vi "Migrate v1 Data.vi"(8 "error in (no error)":errorcluster, 11 "Data Folder":path) -> (0 "error out":errorcluster, 3 "migrated?":bool)   [LabVIEW 2024]
doc: "Converts a version-1 data folder to the schema-version-2 layout (see Documentation/Sample Data/README.md). Does nothing and returns migrated? = FALSE when Projects.ini is missing or already carries [_Meta] Schema Version = 2. Otherwise: (1) every *.ini file is copied into a new subfolder Backup v1 YYYY-MM-DD HHMMSS - if that fails the VI stops with the error and changes nothing; (2) Projects.ini is read: each section except [Default] becomes a project with a new GUID (Active TRUE, Sort Order in file order) and its Task_n keys become tasks with new GUIDs (Active from the ::Active / ::Inactive suffix); [Default] becomes Settings.ini [Default Tasks] Task_0..n; (3) every YYYY-MM.ini month file is read - entries keep their GUID, project and task names are resolved to IDs and missing ones are created with Active FALSE; (4) the version-1 month files are deleted (they are in the backup), Projects.ini and Tasks.ini are written through Project Store-INI and every entry is saved through Time Entry Store-INI, which files it by its UTC Start Time. Stray files such as Projects - Copy.ini are only backed up.\n\nGenerated by: Claude"
uses:
  Project Store-INI/Project Store-INI.lvclass
  Time Entry Store-INI/Time Entry Store-INI.lvclass
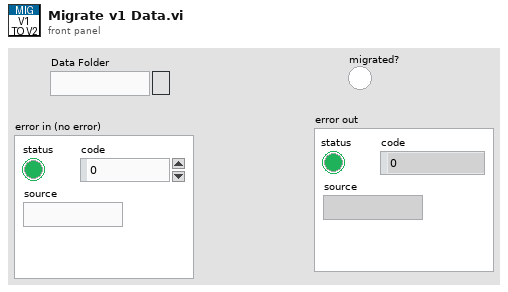
[diagram p1: front panel]
types:
  T1 = typedef "Task List.ctl" = T2[]
  T2 = typedef "Task.ctl" = cluster{"ID":string, "Project ID":string, "Name":string, "Active":bool, "Sort Order":i32}
  T3 = typedef "Project List.ctl" = T4[]
  T4 = typedef "Project.ctl" = cluster{"ID":string, "Name":string, "Active":bool, "Sort Order":i32}
  T5 = cluster{"String":string, "String":string, "String":string, timestamp, timestamp, "String":string}
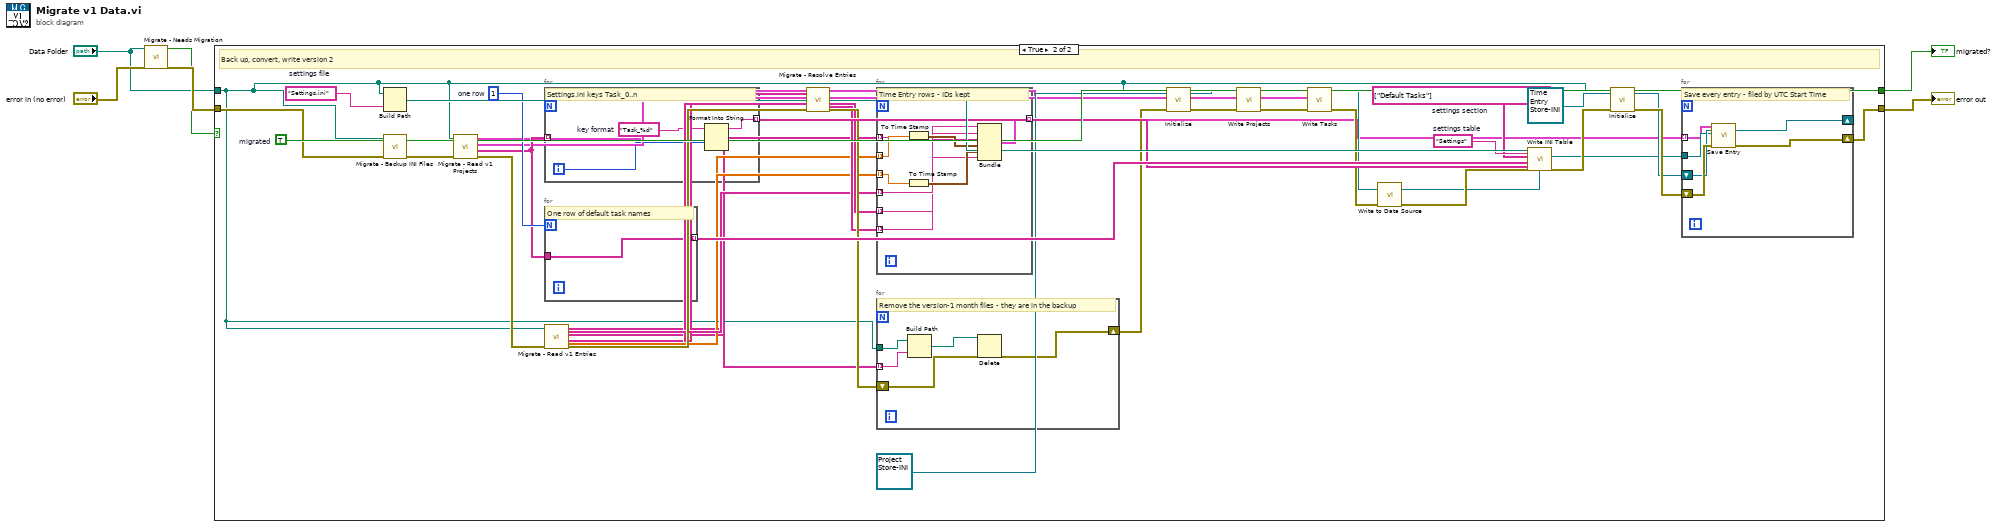
[diagram p0: block diagram]
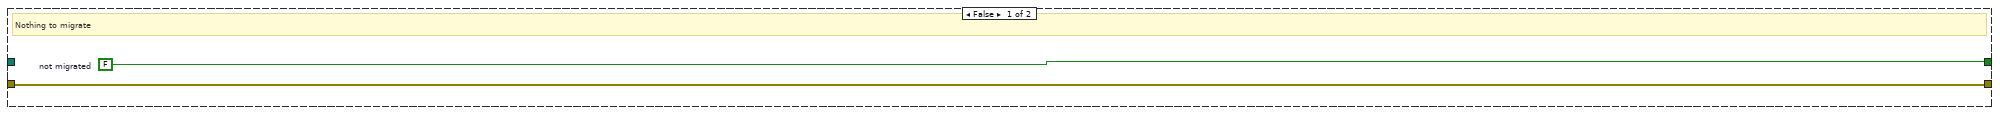
[diagram p2: hidden frame]
diagram:
  n1 = call "Migrate - Needs Migration.vi"("error in (no error)"="error in (no error)", "Data Folder"="Data Folder") -> ("error out"=w4:errorcluster, "needs migration?"=w3:bool)  [unwired: 8 in]
  n2 = case shown="True" w3 {
    tunnel: "Data Folder" -> [_ w9]
    tunnel: [w8 w52] -> w5
    tunnel: w4 -> [w7 w10]
    tunnel: [w7 w51] -> w6
    frame False {
      w8 = FALSE  # not migrated
      # "Nothing to migrate"
    }
    frame True {
      w52 = TRUE  # migrated
      w45 = "Settings.ini"  # settings file
      w44 = "Settings"  # settings table
      w43 = string[] ["Default Tasks"]  # settings section
      w41 = 1  # one row
      # "Back up, convert, write version 2"
      n3 = Build Path(base path=w9, name or relative path=w45) -> (appended path=w46:path)
      n4 = call "Migrate - Backup INI Files.vi"("error in (no error)"=w10, "Data Folder"=w9) -> ("error out"=w11:errorcluster)  [unwired: 8 in, 1 out]
      n5 = call "Migrate - Read v1 Projects.vi"("error in (no error)"=w11, "Data Folder"=w9) -> ("error out"=w15:errorcluster, "Default Task Names"=w14:string[], "Tasks"=w13:T1, "Projects"=w12:T3)  [unwired: 6 in]
      n6 = for {
        tunnel: [w62] -> w40 mode=indexing
        tunnel: w14 -> [_] mode=indexing
        i -> [w60]
        w61 = "Task_%d"  # key format
        # "Settings.ini keys Task_0..n"
        n7 = Format Into String(format string=w61, w60) -> (resulting string=w62:string)  [unwired: 2 in, 1 out]
      }
      n8 = for {
        N: w41 -> [_]
        tunnel: w14 -> [w59]
        tunnel: [w59] -> w42 mode=indexing
        # "One row of default task names"
      }
      n9 = call "Migrate - Read v1 Entries.vi"("error in (no error)"=w15, "Data Folder"=w9) -> ("error out"=w23:errorcluster, "Task Names"=w18:string[], "Entry IDs"=w17:string[], "Month File Names"=w16:string[], "Project Names"=w19:string[], "Descriptions"=w22:string[], "Start Times"=w20:dbl[], "End Times"=w21:dbl[])  [unwired: 2 in]
      n10 = call "Migrate - Resolve Entries.vi"("Task Names"=w18, "error in (no error)"=w23, "Project Names"=w19, "Tasks in"=w13, "Projects in"=w12) -> ("error out"=w28:errorcluster, "Project IDs"=w26:string[], "Tasks out"=w25:T1, "Projects out"=w24:T3, "Task IDs"=w27:string[])  [unwired: 2 in]
      n11 = for {
        tunnel: w17 -> [w68] mode=indexing
        tunnel: w20 -> [w71] mode=indexing
        tunnel: w21 -> [w72] mode=indexing
        tunnel: w22 -> [w73] mode=indexing
        tunnel: w26 -> [w69] mode=indexing
        tunnel: w27 -> [w70] mode=indexing
        tunnel: [w76] -> w29 mode=indexing
        # "Time Entry rows - IDs kept"
        n12 = To Time Stamp(1:w71) -> (0:w74:timestamp)
        n13 = To Time Stamp(1:w72) -> (0:w75:timestamp)
        n14 = Bundle("String"=w68, "String"=w69, "String"=w70, w74, w75, "String"=w73) -> (w76:T5)  [unwired: 1 in]
      }
      n15 = for {
        tunnel: w9 -> [w64]
        tunnel: w16 -> [w63] mode=indexing
        shift-right: [w66] -> w30
        shift-left: w28 -> [w65]
        # "Remove the version-1 month files - they are in the backup"
        n16 = Build Path(base path=w64, name or relative path=w63) -> (appended path=w67:path)
        n17 = Delete(path (use dialog)=w67, error in=w65) -> (error out=w66:errorcluster)  [unwired: 3 in, 2 out]
      }
      n18 = call-dynamic "Initialize.vi"("Project Store in"=refnum<class "Project Store-INI.lvclass"> refnum ("project store"), "error in (no error)"=w30, "Data Folder"=w9) -> ("error out"=w33:errorcluster, "Project Store out"=w32:refnum<class "Project Store-INI.lvclass">)  [unwired: 7 in]
      n19 = call-dynamic "Write Projects.vi"("error in (no error)"=w33, "Project List"=w24, "Project Store in"=w32) -> ("error out"=w34:errorcluster, "Project Store out"=w35:refnum<class "Project Store-INI.lvclass">)  [unwired: 7 in]
      n20 = call-dynamic "Write Tasks.vi"("error in (no error)"=w34, "Task List"=w25, "Project Store in"=w35) -> ("error out"=w36:errorcluster, "Project Store out"=w37:refnum<class "Project Store-INI.lvclass">)  [unwired: 7 in]
      n21 = call-dynamic "Write to Data Source.vi"("Project Store in"=w37, "error in (no error)"=w36) -> ("error out"=w39:errorcluster, "Project Store out"=w38:refnum<class "Project Store-INI.lvclass">)  [unwired: 8 in]
      n22 = call "Write INI Table.vi"("Keys"=w40, "Table Name"=w44, "error in (no error)"=w39, "Values"=w42, "Section Names"=w43, "File Path"=w46) -> ("error out"=w47:errorcluster)  [unwired: 5 in]
      n23 = call-dynamic "Initialize.vi"("Time Entry Store in"=refnum<class "Time Entry Store-INI.lvclass"> refnum ("entry store"), "error in (no error)"=w47, "Data Folder"=w9) -> ("error out"=w50:errorcluster, "Time Entry Store out"=w49:refnum<class "Time Entry Store-INI.lvclass">)  [unwired: 7 in]
      n24 = for {
        tunnel: w29 -> [w53] mode=indexing
        tunnel: w38 -> [w54]
        shift-right: [w56] -> _
        shift-left: w49 -> [w55]
        shift-right: [w58] -> w51
        shift-left: w50 -> [w57]
        # "Save every entry - filed by UTC Start Time"
        n25 = call-dynamic "Save Entry.vi"("Time Entry Store in"=w55, "error in (no error)"=w57, "Project Store"=w54, "Time Entry"=w53) -> ("error out"=w58:errorcluster, "Time Entry Store out"=w56:refnum<class "Time Entry Store-INI.lvclass">)  [unwired: 6 in]
      }
    }
  }
  "migrated?" <- w5
  "error out" <- w6
